vi "HandleItemActivation.vi"(8 "error in (no error)":errorcluster, 11 "RunVI in":refnum<class "RunVI.lvclass">) -> (0 "error out":errorcluster, 3 "RunVI out":refnum<class "RunVI.lvclass">)   [LabVIEW 2023, in "GettingStartedWindow.lvlib" / "RunVI.lvclass"]
uses:
  <resource>/modes/FRC/GSW/Classes/RunVI/RunVI.lvclass
  <resource>/modes/FRC/GSW/Classes/RunVI/RunVI.lvclass/RunVI.ctl
  <resource>/modes/FRC/GSW/GettingStartedWindow.lvlib
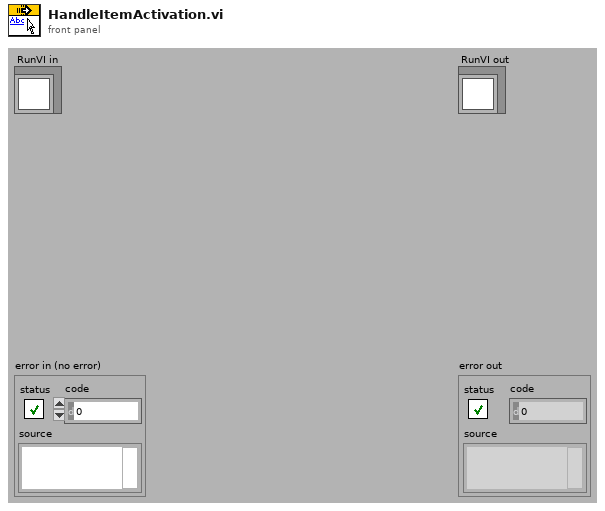
[diagram p1: front panel]
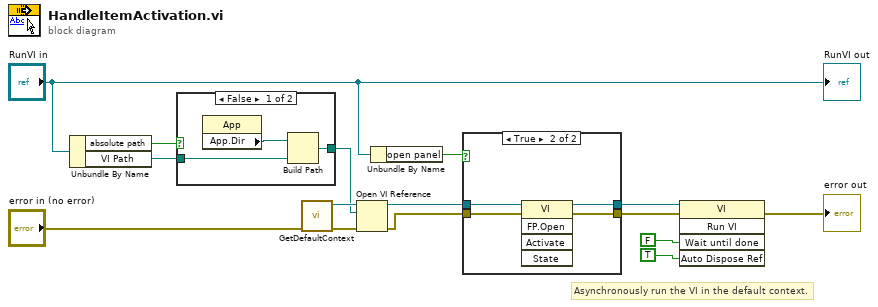
[diagram p0: block diagram]
diagram:
  # "Asynchronously run the VI in the default context."
  n1 = Unbundle By Name("RunVI in") -> ("absolute path"=w7:bool, "VI Path"=w9:path)
  n2 = case shown="False" w7 {
    tunnel: w9 -> [w16 w18]
    tunnel: [w15 w18] -> w8
    frame False {
      n3 = property class="App"() -> ("App.Dir"=w17:path)  [unwired: 2 in, 2 out]
      n4 = Build Path(base path=w17, name or relative path=w16) -> (appended path=w15:path)
    }
    frame True {
    }
  }
  n5 = call <resource>:"GetDefaultContext.vi"() -> ("Context"=w14:refnum<vi>)  [unwired: 11 in]
  n6 = Open VI Reference(application reference (local)=w14, vi path=w8, error in (no error)="error in (no error)") -> (vi reference=w6:refnum<vi>, error out=w4:errorcluster)  [unwired: 3 in]
  n7 = Unbundle By Name("RunVI in") -> ("open panel"=w1:bool)
  n8 = case shown="True" w1 {
    tunnel: w6 -> [w20 w24]
    tunnel: [w20 w23] -> w5
    tunnel: w4 -> [w19 w22]
    tunnel: [w19 w21] -> w3
    frame False {
    }
    frame True {
      n9 = invoke class="VI" method="FP.Open"(reference=w24, error in=w22) -> (reference out=w23:refnum<vi>, error out=w21:errorcluster)  [unwired: 3 in, 3 out]
    }
  }
  n10 = invoke class="VI" method="Run VI"(reference=w5, error in=w3, "Wait until done"=FALSE ("Wait Until Done"), "Auto Dispose Ref"=TRUE ("Auto Dispose Reference")) -> (error out=→"error out":errorcluster)  [unwired: 1 in, 4 out]
  "RunVI out" <- "RunVI in"
